vi "PicoLogCM3Example.vi"() -> ()   [LabVIEW 2010]
panel:
  in  "Stop":bool
  out "End time":timestamp=timestamp(-9593251200 s since 1904-01-01)
  out "Start time":timestamp=timestamp(-9593251200 s since 1904-01-01)
  out "Ch3 Status":enum32{"Red", "Yellow", "Green"}(radio)=enum."Yellow"
  out "Ch2 Status":enum32{"Red", "Yellow", "Green"}(radio)=enum."Yellow"
  out "Ch1 Status":enum32{"Red", "Yellow", "Green"}(radio)=enum."Green"
  out "GetValue PICO_STATUS log":T1(array[cluster]) {"Hex Code" format="%x"}
  in  "CH3 Measurement Type":u32(ring) items=["OFF", "1mV range (1mV/A)", "10mV range (10mV/A)", "100mV range (100mV/A)", "Voltage Input"]
  in  "CH2 Measurement Type":u32(ring) items=["OFF", "1mV range (1mV/A)", "10mV range (10mV/A)", "100mV range (100mV/A)", "Voltage Input"]
  in  "CH1 Measurement Type":u32(ring)=1 items=["OFF", "1mV range (1mV/A)", "10mV range (10mV/A)", "100mV range (100mV/A)", "Voltage Input"]
  out "Unit Info":T2
  in  "IP Address:port number":string="192.168.1.30:6250"
  in  "Enumerate USB/Ethernet/ALL":u32(ring)=4294967295 items=["USB"=1, "Ethernet"=2, "ALL"=4294967295]
  out "plcm3 Units":string
  in  "Connection":bool=TRUE
  in  "Use Serial Number":bool
  in  "Serial Number":string
  out "Chan3 Value":dbl(knob) scale=0.0..100.0
  out "Chan2 Value":dbl(knob) scale=0.0..10.0
  out "Chan1 Value":dbl(knob) max=100.0 scale=0.0..1000.0
  in  "Update settings":bool
  # "USB"
  # "Ethernet"
  # "Channel 1"
  # "Channel 2"
  # "Channel 3"
  # "Channel Status LED-\nYellow- Waiting/Off\nGreen- Read OK\nRed- Read Error"
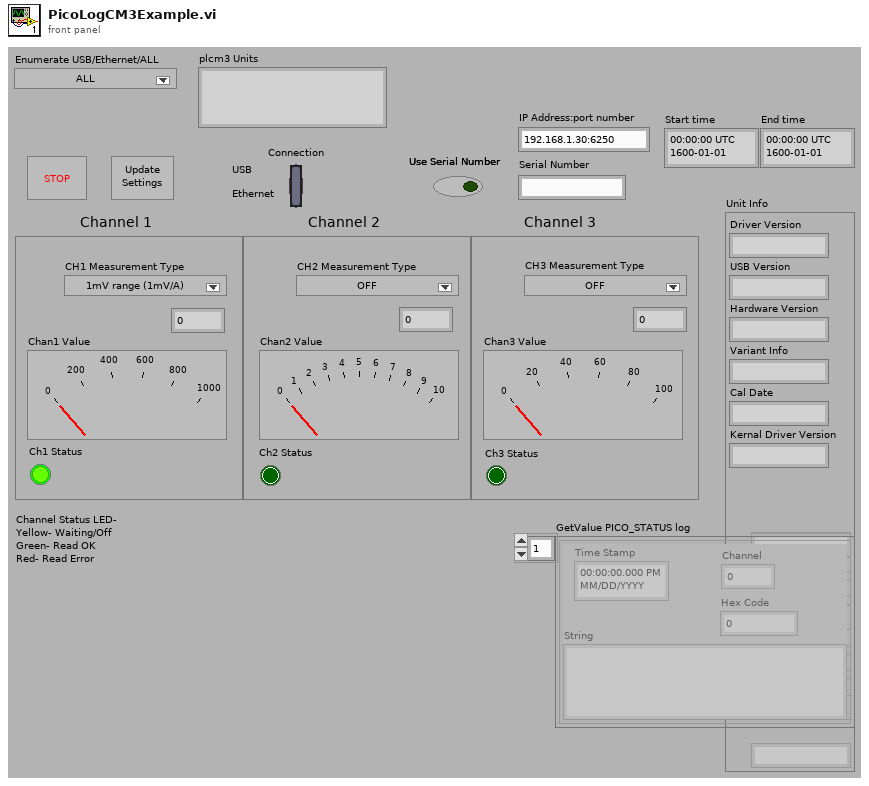
[diagram p1: front panel]
types:
  T1 = cluster{"Time Stamp":timestamp, "Hex Code":i32, "String":string, "Channel":i32}[]
  T2 = cluster{"Driver Version":string, "USB Version":string, "Hardware Version":string, "Variant Info":string, "Cal Date":string, "Kernal Driver Version":string, "NA":string, "NA 2":string, "NA":string, "NA 3":string, "NA 4":string, "NA 5":string, "NA 6":string, "NA 7":string, "NA 8":string}
  T3 = cluster{"seconds since 1Jan1904":timestamp, i32, "String":string, i32}[]
  T4 = cluster{"status":bool, "code":u32, "source":string}
  T5 = cluster{"seconds since 1Jan1904":timestamp, "code":u32, "String":string, i32}
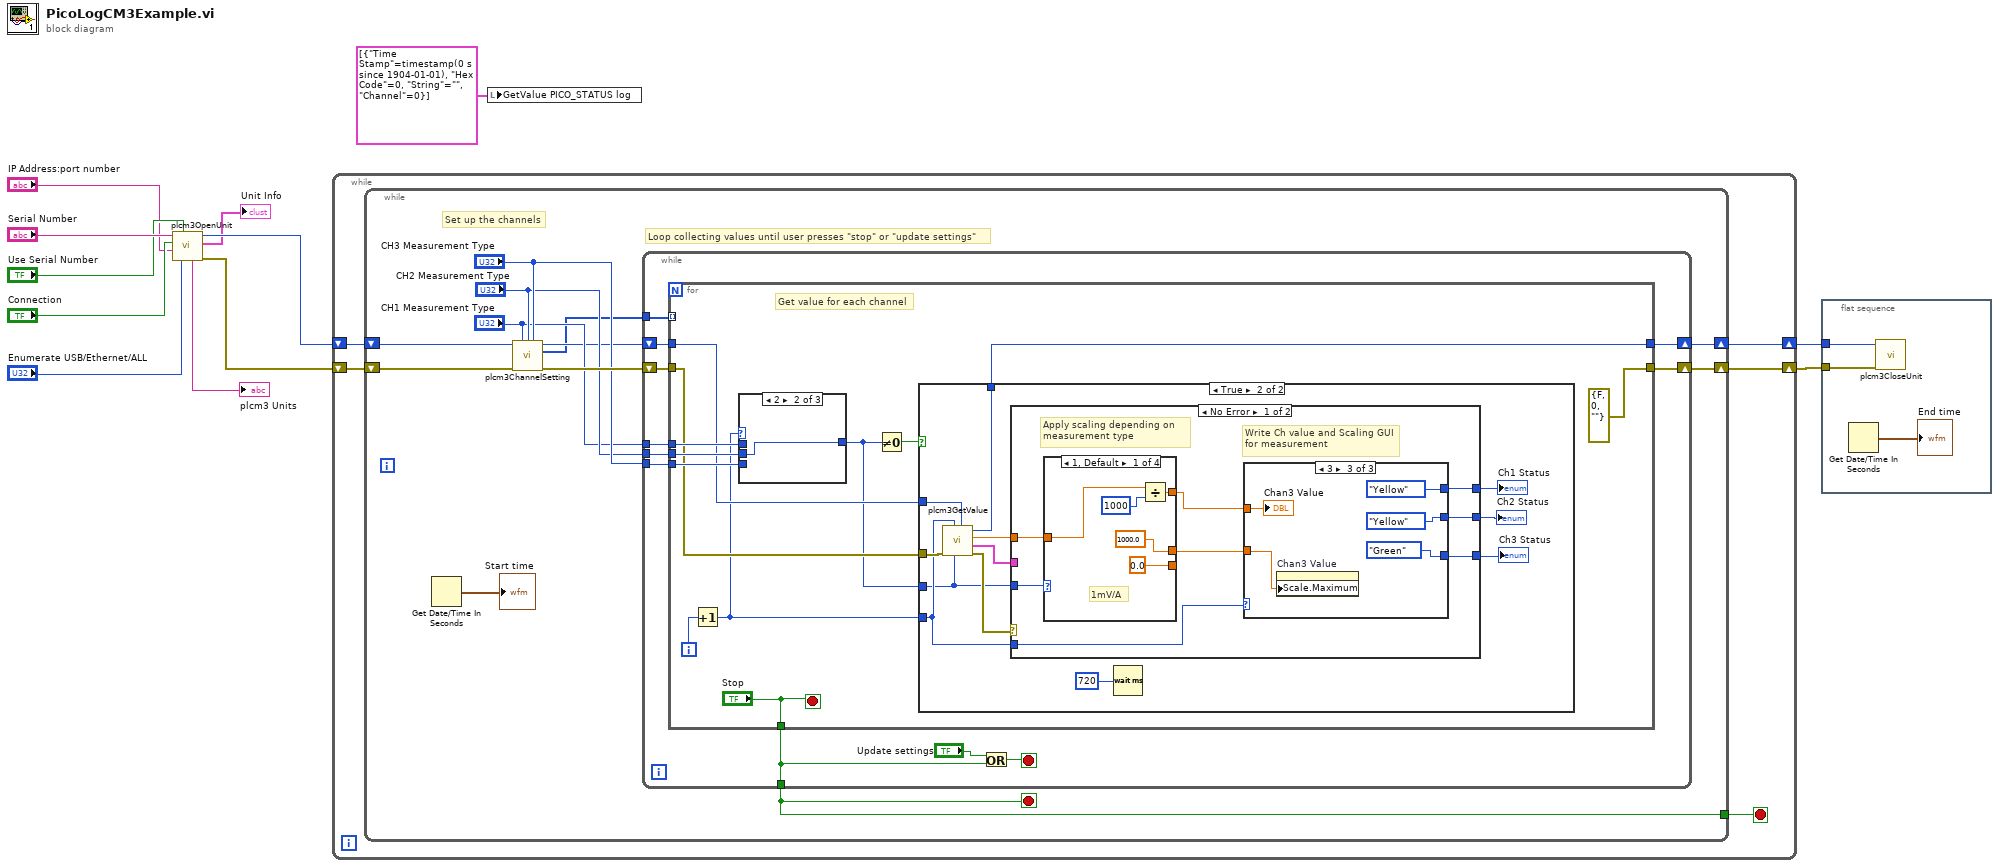
[diagram p0: block diagram]
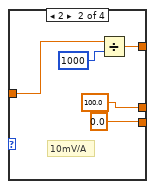
[diagram p3: hidden frame]
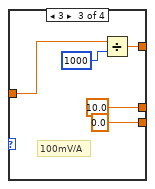
[diagram p4: hidden frame]
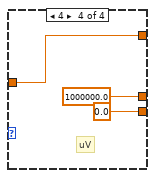
[diagram p5: hidden frame]
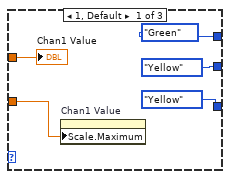
[diagram p6: hidden frame]
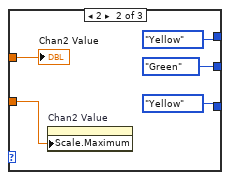
[diagram p7: hidden frame]
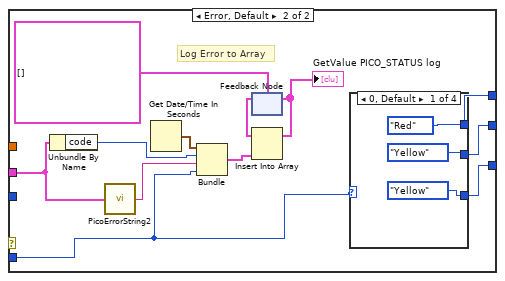
[diagram p8: hidden frame]
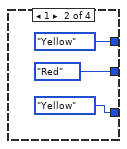
[diagram p9: hidden frame]
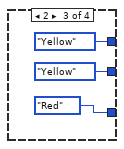
[diagram p10: hidden frame]
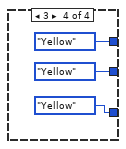
[diagram p11: hidden frame]
diagram:
  n1 = call "plcm3OpenUnit.vi"("IP Address:port number"="IP Address:port number", "Serial Number"="Serial Number", "Use Serial Number"="Use Serial Number", "Enumerate USB/Ethernet/ALL"="Enumerate USB/Ethernet/ALL", "Connection"="Connection") -> ("error out"=w4:errorcluster, "Unit Info"=→"Unit Info":T2, "handle out"=w12:i16, "plcm3 Units"=→"plcm3 Units":string)  [unwired: 2 in, 1 out]
  n2 = while {
    shift-right: [w14] -> w2
    shift-left: w12 -> [w17]
    shift-right: [w15] -> w3
    shift-left: w4 -> [w16]
    stop <- w13 stop-if-true
    n3 = while {
      shift-right: [w26] -> w15
      shift-left: w16 -> [w27]
      shift-right: [w22] -> w14
      shift-left: w17 -> [w29]
      tunnel: [w19] -> w13
      stop <- w19 stop-if-true
      # "Loop collecting values until user presses \"stop\" or \"update settings\""
      # "Set up the channels"
      n4 = Get Date/Time In Seconds() -> (seconds since 1Jan1904=→"Start time":timestamp)
      n5 = call "plcm3ChannelSetting.vi"("Handle In"=w29, "CH1 Measurement Type"="CH1 Measurement Type", "CH2 Measurement Type"="CH2 Measurement Type", "CH3 Measurement Type"="CH3 Measurement Type", "error in (no error)"=w27) -> ("Handle out"=w21:i16, "Channel Enable Array"=w18:u8[], "error out"=w28:errorcluster)  [unwired: 8 in]
      n6 = while {
        tunnel: "CH1 Measurement Type" -> [w37]
        tunnel: "CH2 Measurement Type" -> [w36]
        tunnel: "CH3 Measurement Type" -> [w35]
        shift-right: [w39] -> w26
        shift-left: w28 -> [w40]
        shift-right: [w38] -> w22
        shift-left: w21 -> [w34]
        tunnel: [w32] -> w19
        tunnel: w18 -> [w30]
        stop <- w33 stop-if-true
        n7 = for {
          tunnel: w40 -> [w49]
          tunnel: w34 -> [w48]
          tunnel: [errorcluster {"status"=FALSE, "code"=0, "source"=""} ("error out")] -> w39
          tunnel: [w47] -> w38
          tunnel: w37 -> [w52]
          tunnel: w36 -> [w51]
          tunnel: w35 -> [w50]
          tunnel: ["Stop"] -> w32
          tunnel: w30 -> [_] mode=indexing
          i -> [w42]
          stop <- "Stop" stop-if-true
          # "Get value for each channel"
          n8 = Increment(x=w42) -> (x+1=w46:i32)
          n9 = case shown="2" w46 {
            tunnel: [w131 w132 w133] -> w44
            tunnel: w52 -> [w131 _ _]
            tunnel: w51 -> [_ w132 _]
            tunnel: w50 -> [_ _ w133]
            frame 1, Default {
            }
            frame 2 {
            }
            frame 3 {
            }
          }
          n10 = Not Equal To 0?(x=w44) -> (x != 0?=w45:bool)
          n11 = case shown="True" w45 {
            tunnel: w49 -> [_ w65]
            tunnel: w48 -> [w53 w64]
            tunnel: [w53 w63] -> w47
            tunnel: w46 -> [_ w59]
            tunnel: w44 -> [_ w55]
            frame False {
            }
            frame True {
              n12 = call "plcm3GetValue.vi"("Measurement Type"=w55, "Channel"=w59, "error in (no error)"=w65, "handle in"=w64) -> ("error out"=w57:errorcluster, "PICO_STATUS out"=w54:T4, "Channel Data"=w58:dbl, "handle out"=w63:i16)  [unwired: 4 in]
              n13 = case shown="No Error" w57 {
                tunnel: w58 -> [w69 _]
                tunnel: w59 -> [w73 w112]
                tunnel: [w72 w114] -> w62
                tunnel: [w71 w113] -> w61
                tunnel: [w70 w111] -> w60
                tunnel: w55 -> [w67 _]
                tunnel: w54 -> [_ w107]
                frame No Error {
                  # "Apply scaling depending on \nmeasurement type"
                  # "Write Ch value and Scaling GUI for measurement"
                  n14 = case shown="1, Default" w67 {
                    tunnel: w69 -> [w77 w82 w87 w89]
                    tunnel: [w76 w81 w86 w89] -> w68
                    tunnel: [1000.0 ("Data Range:Maximum") 100.0 ("Data Range:Maximum") 10.0 ("Data Range:Maximum") 1000000.0 ("Data Range:Maximum")] -> w66
                    tunnel: [0.0 ("Scale.Range:Minimum") 0.0 ("Scale.Range:Minimum") 0.0 ("Scale.Range:Minimum") 0.0 ("Scale.Range:Minimum")] -> _
                    frame 1, Default {
                      # "1mV/A"
                      n15 = Divide(x=w77, y=1000) -> (x/y=w76:dbl)
                    }
                    frame 2 {
                      # "10mV/A"
                      n16 = Divide(x=w82, y=1000) -> (x/y=w81:dbl)
                    }
                    frame 3 {
                      # "100mV/A"
                      n17 = Divide(x=w87, y=1000) -> (x/y=w86:dbl)
                    }
                    frame 4 {
                      # "uV"
                    }
                  }
                  n18 = case shown="3" w73 {
                    tunnel: w68 -> [w93 w98 w103]
                    tunnel: [enum32{"Red", "Yellow", "Green"}."Green" ("Select") enum32{"Red", "Yellow", "Green"}."Yellow" ("Select") enum32{"Red", "Yellow", "Green"}."Yellow" ("Select")] -> w72
                    tunnel: [enum32{"Red", "Yellow", "Green"}."Yellow" ("Select") enum32{"Red", "Yellow", "Green"}."Green" ("Select") enum32{"Red", "Yellow", "Green"}."Yellow" ("Select")] -> w71
                    tunnel: [enum32{"Red", "Yellow", "Green"}."Yellow" ("Select") enum32{"Red", "Yellow", "Green"}."Yellow" ("Select") enum32{"Red", "Yellow", "Green"}."Green" ("Select")] -> w70
                    tunnel: w66 -> [w92 w97 w102]
                    frame 1, Default {
                      n19 = property on="Chan1 Value" class="Knob (strict)"("Scale.Maximum"=w92) -> ()  [unwired: 2 in, 2 out]
                      "Chan1 Value" <- w93
                    }
                    frame 2 {
                      n20 = property on="Chan2 Value" class="Knob (strict)"("Scale.Maximum"=w97) -> ()  [unwired: 2 in, 2 out]
                      "Chan2 Value" <- w98
                    }
                    frame 3 {
                      n21 = property on="Chan3 Value" class="Knob (strict)"("Scale.Maximum"=w102) -> ()  [unwired: 2 in, 2 out]
                      "Chan3 Value" <- w103
                    }
                  }
                }
                frame Error, Default {
                  # "Log Error to Array"
                  n22 = Unbundle By Name(w107) -> ("code"=w108:u32)
                  n23 = call "PicoErrorString2.vi"("PICO_STATUS in"=w107) -> ("String"=w109:string)  [unwired: 2 in, 2 out]
                  n24 = Get Date/Time In Seconds() -> (seconds since 1Jan1904=w115:timestamp)
                  n25 = Bundle("seconds since 1Jan1904"=w115, "code"=w108, "String"=w109, w112) -> (w118:T5)  [unwired: 1 in]
                  n26 = feedback #1(T3 []) -> (w116:T3)
                  n27 = Insert Into Array(array=w116, new element=w118) -> (w117:T3)  [unwired: 1 in]
                  "GetValue PICO_STATUS log" <- w117
                  n28 = feedback-in #1(w117) -> ()
                  n29 = case shown="0, Default" w112 {
                    tunnel: [enum32{"Red", "Yellow", "Green"}."Red" ("Select") enum32{"Red", "Yellow", "Green"}."Yellow" ("Select") enum32{"Red", "Yellow", "Green"}."Yellow" ("Select") enum32{"Red", "Yellow", "Green"}."Yellow" ("Select")] -> w114
                    tunnel: [enum32{"Red", "Yellow", "Green"}."Yellow" ("Select") enum32{"Red", "Yellow", "Green"}."Red" ("Select") enum32{"Red", "Yellow", "Green"}."Yellow" ("Select") enum32{"Red", "Yellow", "Green"}."Yellow" ("Select")] -> w113
                    tunnel: [enum32{"Red", "Yellow", "Green"}."Yellow" ("Select") enum32{"Red", "Yellow", "Green"}."Yellow" ("Select") enum32{"Red", "Yellow", "Green"}."Red" ("Select") enum32{"Red", "Yellow", "Green"}."Yellow" ("Select")] -> w111
                    frame 0, Default {
                    }
                    frame 1 {
                    }
                    frame 2 {
                    }
                    frame 3 {
                    }
                  }
                }
              }
              "Ch1 Status" <- w62
              "Ch2 Status" <- w61
              "Ch3 Status" <- w60
              n30 = Wait (ms)(milliseconds to wait=u32 720) -> ()  [unwired: 1 out]
            }
          }
        }
        n31 = Or(x="Update settings", y=w32) -> (x .or. y?=w33:bool)
      }
    }
  }
  n32 = local write "GetValue PICO_STATUS log"(T1 [{"Time Stamp"=timestamp(0 s since 1904-01-01), "Hex Code"=0, "String"="", "Channel"=0}] ("GetValue PICO_STATUS log")) -> ()
  n33 = flat-sequence {
    tunnel: w3 -> [w136]
    tunnel: w2 -> [w135]
    frame #0 {
      n34 = Get Date/Time In Seconds() -> (seconds since 1Jan1904=→"End time":timestamp)
      n35 = call "plcm3CloseUnit.vi"("error in (no error)"=w136, "handle in"=w135) -> ()  [unwired: 8 in, 2 out]
    }
  }
